vi "BSD Data accumlation.vi"(5 "Assigned#_CL":T2, 6 "LSPX_C1":T4, 7 "LCPX_CZ":T1, 8 "error in (no error)":errorcluster caption="error in", 9 "LSP_C2 before":T2, 10 "LSP_C1 before":T3, 11 "LCPZ before":T1) -> (0 "error out":errorcluster, 1 "LSP_C2 after":T2, 2 "LSP_C1 after":T3, 3 "LCPZ after":T1)   [LabVIEW 2018]
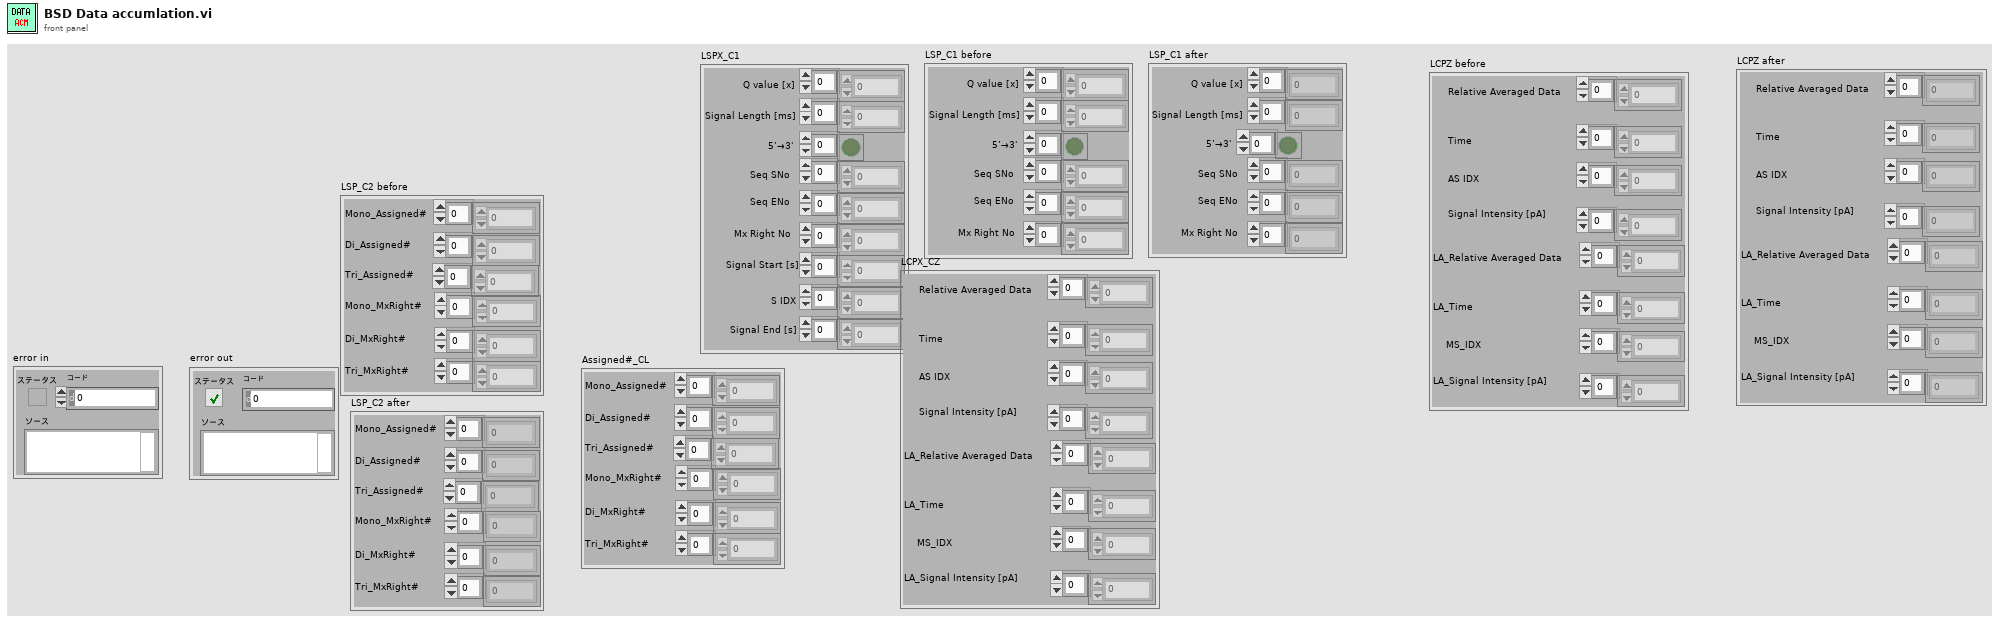
[diagram p1: front panel]
types:
  T1 = cluster{"Relative Averaged Data":dbl[], "Time":dbl[], "AS IDX":i32[], "Signal Intensity [pA]":dbl[], "LA_Relative Averaged Data":dbl[], "LA_Time":dbl[], "MS_IDX":i32[], "LA_Signal Intensity [pA]":dbl[]}
  T2 = cluster{"Mono_Assigned#":i32[], "Di_Assigned#":i32[], "Tri_Assigned#":i32[], "Tri_MxRight#":i32[], "Di_MxRight#":i32[], "Mono_MxRight#":i32[]}
  T3 = cluster{"Q value [x]":dbl[], "Signal Length [ms]":dbl[], "5’→3'":bool[], "Seq SNo":i32[], "Seq ENo":i32[], "Mx Right No":i32[]}
  T4 = cluster{"Q value [x]":dbl[], "Signal Length [ms]":dbl[], "5’→3'":bool[], "Seq SNo":i32[], "Seq ENo":i32[], "Mx Right No":i32[], "Signal Start [s]":dbl[], "S IDX":i32[], "Signal End [s]":dbl[]}
  T5 = cluster{dbl[], dbl[], i32[], dbl[], dbl[], dbl[], i32[], dbl[]}
  T6 = cluster{dbl[], dbl[], bool[], i32[], i32[], i32[]}
  T7 = cluster{i32[], i32[], i32[], i32[], i32[], i32[]}
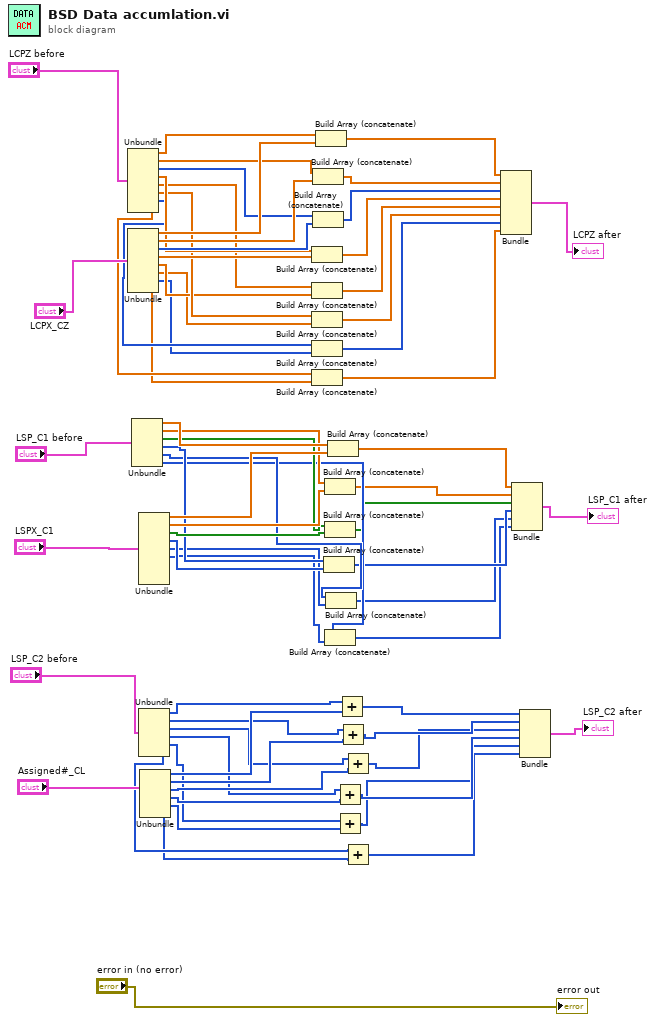
[diagram p0: block diagram]
diagram:
  n1 = Unbundle("LCPZ before") -> ("Relative Averaged Data"=w70:dbl[], "Time"=w68:dbl[], "AS IDX"=w66:i32[], "Signal Intensity [pA]"=w64:dbl[], "LA_Relative Averaged Data"=w12:dbl[], "LA_Time"=w11:dbl[], "MS_IDX"=w10:i32[], "LA_Signal Intensity [pA]"=w9:dbl[])
  n2 = Unbundle("LCPX_CZ") -> ("Relative Averaged Data"=w69:dbl[], "Time"=w67:dbl[], "AS IDX"=w65:i32[], "Signal Intensity [pA]"=w63:dbl[], "LA_Relative Averaged Data"=w8:dbl[], "LA_Time"=w7:dbl[], "MS_IDX"=w6:i32[], "LA_Signal Intensity [pA]"=w5:dbl[])
  n3 = Unbundle("LSP_C1 before") -> ("Q value [x]"=w62:dbl[], "Signal Length [ms]"=w60:dbl[], "5’→3'"=w58:bool[], "Seq SNo"=w56:i32[], "Seq ENo"=w54:i32[], "Mx Right No"=w52:i32[])
  n4 = Unbundle("LSPX_C1") -> ("Q value [x]"=w61:dbl[], "Signal Length [ms]"=w59:dbl[], "5’→3'"=w57:bool[], "Seq SNo"=w55:i32[], "Seq ENo"=w53:i32[], "Mx Right No"=w51:i32[])  [unwired: 3 out]
  n5 = Unbundle("LSP_C2 before") -> ("Mono_Assigned#"=w33:i32[], "Di_Assigned#"=w30:i32[], "Tri_Assigned#"=w27:i32[], "Tri_MxRight#"=w24:i32[], "Di_MxRight#"=w21:i32[], "Mono_MxRight#"=w18:i32[])
  n6 = Unbundle("Assigned#_CL") -> ("Mono_Assigned#"=w32:i32[], "Di_Assigned#"=w29:i32[], "Tri_Assigned#"=w26:i32[], "Tri_MxRight#"=w23:i32[], "Di_MxRight#"=w20:i32[], "Mono_MxRight#"=w17:i32[])
  n7 = Build Array (concatenate)(w64, w63) -> (w47:dbl[])
  n8 = Build Array (concatenate)(w12, w8) -> (w4:dbl[])
  n9 = Build Array (concatenate)(w11, w7) -> (w3:dbl[])
  n10 = Build Array (concatenate)(w10, w6) -> (w2:i32[])
  n11 = Build Array (concatenate)(w9, w5) -> (w1:dbl[])
  n12 = Build Array (concatenate)(w68, w67) -> (w49:dbl[])
  n13 = Build Array (concatenate)(w66, w65) -> (w48:i32[])
  n14 = Build Array (concatenate)(w70, w69) -> (w50:dbl[])
  n15 = Build Array (concatenate)(w56, w55) -> (w43:i32[])
  n16 = Build Array (concatenate)(w60, w59) -> (w45:dbl[])
  n17 = Build Array (concatenate)(w58, w57) -> (w44:bool[])
  n18 = Build Array (concatenate)(w52, w51) -> (w41:i32[])
  n19 = Build Array (concatenate)(w54, w53) -> (w42:i32[])
  n20 = Build Array (concatenate)(w62, w61) -> (w46:dbl[])
  n21 = Add(x=w24, y=w23) -> (x+y=w22:i32[])
  n22 = Add(x=w21, y=w20) -> (x+y=w19:i32[])
  n23 = Add(x=w33, y=w32) -> (x+y=w31:i32[])
  n24 = Add(x=w30, y=w29) -> (x+y=w28:i32[])
  n25 = Add(x=w27, y=w26) -> (x+y=w25:i32[])
  n26 = Add(x=w18, y=w17) -> (x+y=w16:i32[])
  n27 = Bundle(w50, w49, w48, w47, w4, w3, w2, w1) -> (→"LCPZ after":T5)  [unwired: 1 in]
  n28 = Bundle(w46, w45, w44, w43, w42, w41) -> (→"LSP_C1 after":T6)  [unwired: 1 in]
  n29 = Bundle(w31, w28, w25, w22, w19, w16) -> (→"LSP_C2 after":T7)  [unwired: 1 in]
  "error out" <- "error in (no error)"
